vi "Prepare.vi"(8 "error in (no error)":errorcluster, 11 "CIFPlugin in":refnum<class "CAN_Writer_CANsub_Plugin.lvclass">) -> (0 "error out":errorcluster, 3 "CIFPlugin out":refnum<class "CAN_Writer_CANsub_Plugin.lvclass">)   [LabVIEW 2021, in "CAN_Writer_CANsub_Plugin.lvclass"]
uses:
  CAN_Writer_CANsub_Plugin.lvclass
  CAN_Writer_CANsub_Plugin.lvclass/CAN_Writer_CANsub_Plugin.ctl
  <vilib>/CIF Foundation/CIF XNET CAN RW/XNET CAN RW.lvclass
  <vilib>/CIF Foundation/CIF CAN RW Core/CAN_RW_CORE.lvclass
  <vilib>/CIF Foundation/CIF Core/CIFCore/Common/Typedef/Multi_Cycle Logic State Enum.ctl
  <vilib>/CIF Foundation/CIF Core/CIFCore/Common/CIFCoreCommon.lvlib
  Typedef/Internal Data.ctl
  <vilib>/CIF Foundation/CIF Core/CIFCore/Common/Typedef/FIFO Drop Internal Data.ctl
  C:/Program Files/National Instruments/LabVIEW 2021/vi.lib/CIF Foundation/CIF CAN RW Core/CAN_RW_CORE.lvclass
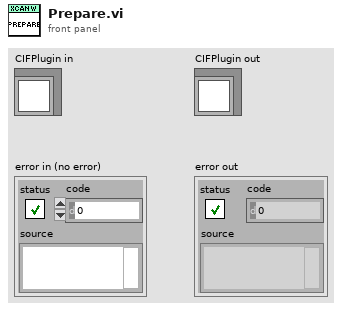
[diagram p1: front panel]
types:
  T1 = typedef "CAN_Writer_CANsub_Plugin.lvclass/Internal Data.ctl" = cluster{"Logic State Enum":T2, "FIFO Drop":T3}
  T2 = typedef "CIFCoreCommon.lvlib/Multi_Cycle Logic State Enum.ctl" = enum16{"Read FIFO", "Sleep", "Output Data"}
  T3 = typedef "CIFCoreCommon.lvlib/FIFO Drop Internal Data.ctl" = cluster{"Last FIFO Ctr":u64, "FIFO Ctr Valid":bool}
  T4 = typedef "CAN_RW_CORE.lvclass/CAN Port Configuration.ctl" = cluster{"Mode":T5, "Baud Rate":u64, "Temination On":bool, "Subordinate":bool, "Echo TX":bool, "FD Config":T6}
  T5 = typedef "CAN_RW_CORE.lvclass/CAN Mode.ctl" = enum16{"CAN 2.0", "CAN FD"}
  T6 = typedef "CAN_RW_CORE.lvclass/FD Config.ctl" = cluster{"FD Baud Rate":u64, "ISO Mode":bool, "BRS Enabled":bool}
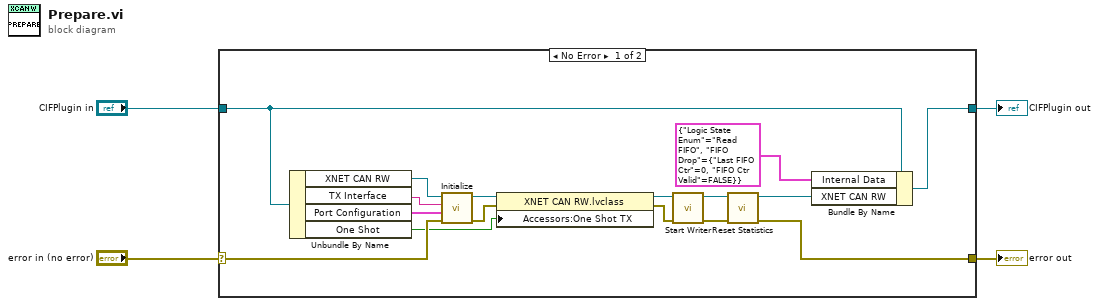
[diagram p0: block diagram]
diagram:
  n1 = case shown="No Error" "error in (no error)" {
    selector: "error in (no error)" -> [w17 w22]
    tunnel: [w11 w22] -> w3
    tunnel: [w15 w21] -> w1
    tunnel: "CIFPlugin in" -> [w16 w21]
    frame No Error {
      n2 = Unbundle By Name(w16) -> ("XNET CAN RW"=w20:refnum<class "XNET CAN RW.lvclass">, "TX Interface"=w19:string, "Port Configuration"=w18:T4, "One Shot"=w5:bool)
      n3 = call <vilib>:"Initialize.vi"("error in (no error)"=w17, "Port Configuration"=w18, "Interface"=w19, "XNET_CAN_RW in"=w20) -> ("error out"=w6:errorcluster, "XNET_CAN_RW out"=w9:refnum<class "XNET CAN RW.lvclass">)  [unwired: 6 in]
      n4 = property class="XNET CAN RW.lvclass"(reference=w9, error in=w6, "Accessors:One Shot TX"=w5) -> (reference out=w8:refnum<class "XNET CAN RW.lvclass">, error out=w7:errorcluster)
      n5 = call-dynamic "Start Writer.vi"("error in (no error)"=w7, "XNET_CAN_RW in"=w8) -> ("error out"=w13:errorcluster, "XNET_CAN_RW out"=w14:refnum<class "XNET CAN RW.lvclass">)  [unwired: 8 in]
      n6 = call <vilib>:"Reset Statistics.vi"("error in (no error)"=w13, "CAN_RW_CORE in"=w14) -> ("error out"=w11:errorcluster, "CAN_RW_CORE out"=w12:refnum<class "XNET CAN RW.lvclass">)  [unwired: 8 in]
      n7 = Bundle By Name(cluster=w16, "Internal Data"=T1 {"Logic State Enum"=enum."Read FIFO", "FIFO Drop"={"Last FIFO Ctr"=0, "FIFO Ctr Valid"=FALSE}}, "XNET CAN RW"=w12) -> (w15:refnum<class "CAN_Writer_CANsub_Plugin.lvclass">)
    }
    frame Error {
    }
  }
  "error out" <- w3
  "CIFPlugin out" <- w1
